vi "CreateMeanderMask_3d.vi"(7 "Rep. Rate (Hz)":dbl=10.0 min=0.0 max=34.0, 10 "Start Position":dbl[](array[numeric]) min=0.0 max=34.0) -> (0 "Laser_Ctrl":bool, 1 "start/end points":cluster{dbl, dbl, dbl}[][](array[cluster]), 2 "Canceled":bool, 5 "ImageParameter":T1)   [LabVIEW 2013]
uses:
  ImagingMS/ImageConvPara.ctl
panel:
  in  "Z Steps":i32=1 min=0 max=34
  in  "Z StepWidth":dbl=0.0001 min=0.0 max=34.0
  in  "Apply":bool
  in  "X StepWidth":dbl=0.025 min=0.0 max=34.0
  in  "Imaging?":bool=TRUE
  out "Estimated Time (min)":dbl min=0.0 max=34.0
  in  "Average/pixel":i32=10 min=0 max=34
  in  "Cancel":bool
  in  "Run":bool
  out "XY Graph":cluster{dbl, dbl, "X StepWidth":dbl}[](graph)
  out "Y Size (mm)":dbl min=0.0 max=34.0
  out "X Size (mm)":dbl min=0.0 max=34.0
  in  "Y Steps":i32=64 min=0 max=34
  in  "X Steps":i32=128 min=0 max=34
  in  "Y StepWidth":dbl=0.025 min=0.0 max=34.0
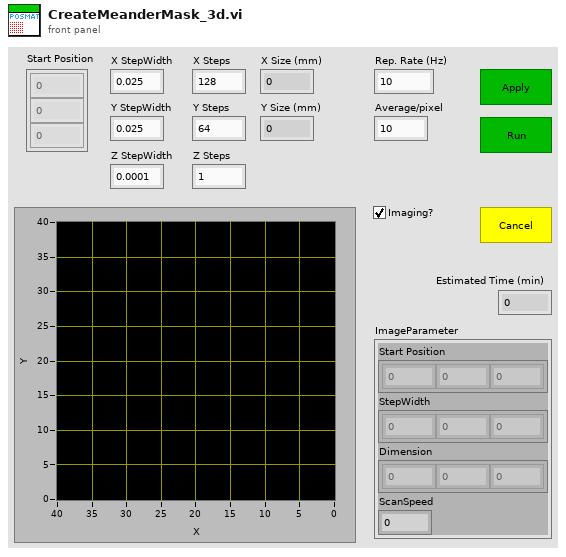
[diagram p1: front panel]
types:
  T1 = typedef "ImageConvPara.ctl" = cluster{"Start Position":dbl[], "StepWidth":dbl[], "Dimension":i32[], "ScanSpeed":dbl}
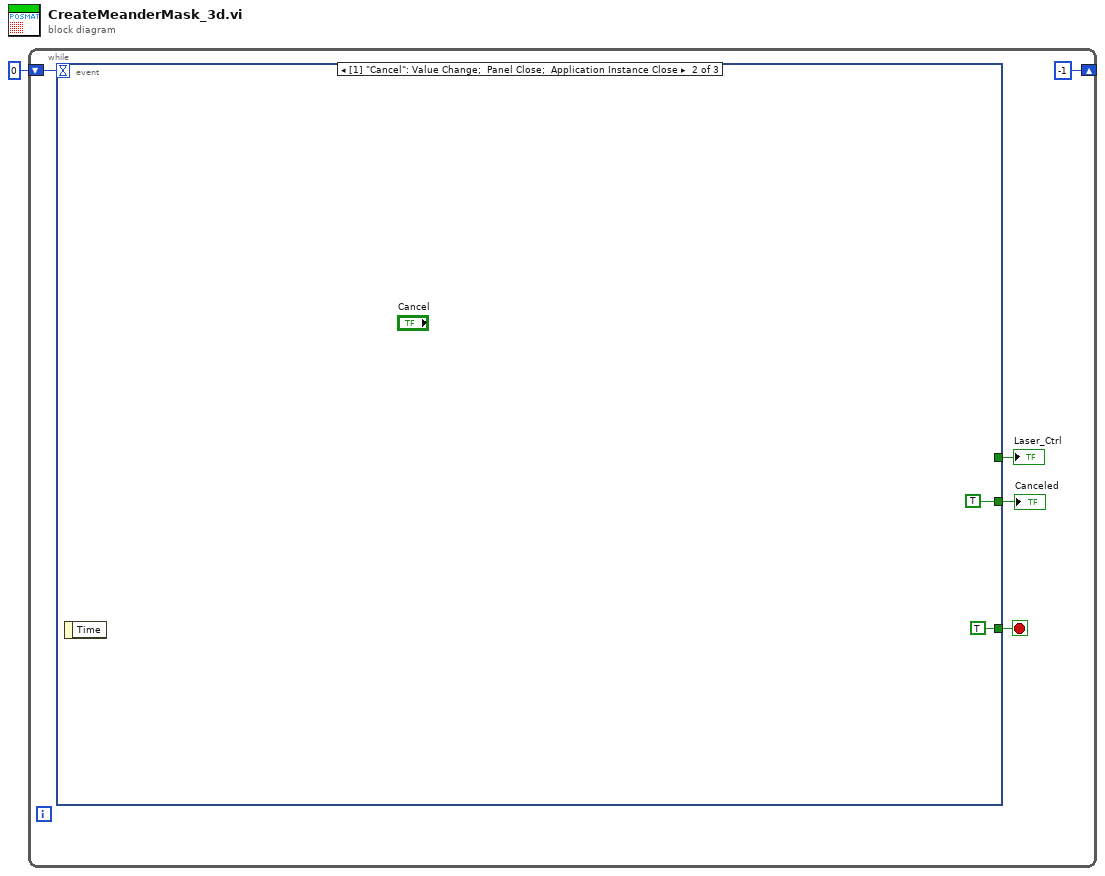
[diagram p0: block diagram]
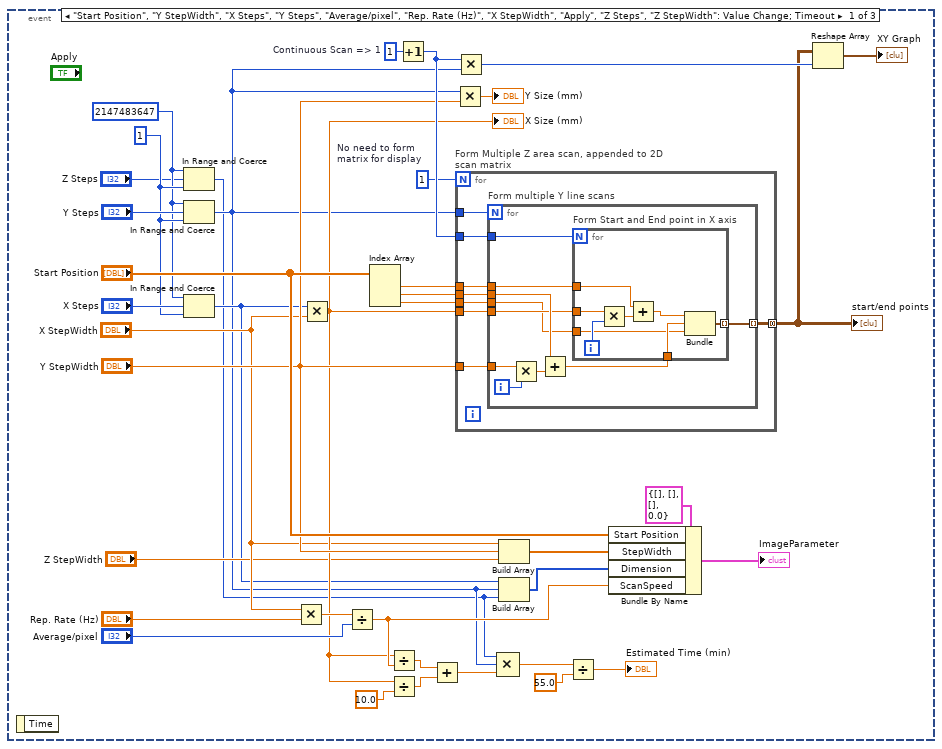
[diagram p2: hidden frame]
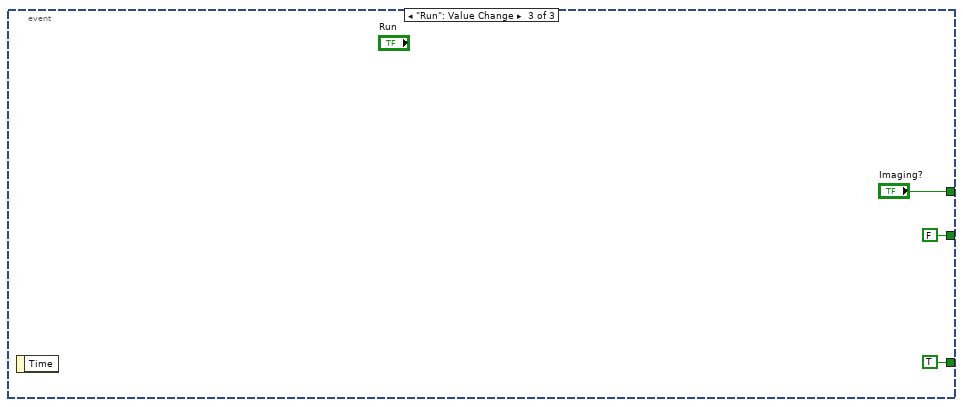
[diagram p3: hidden frame]
diagram:
  n1 = while {
    shift-right: [-1] -> _
    shift-left: 0 -> [w3]
    stop <- w6 stop-if-true
    n2 = event shown="[1] \"Cancel\": Value Change;  Panel Close;  Application Instance Close" {
      selector: _ -> [_ _ _]
      dyn-events: _ -> [_ _ _]
      timeout: w3 -> [_ _ _]
      tunnel: [_ TRUE TRUE] -> w6
      tunnel: [_ TRUE ("Canceled") FALSE ("Canceled")] -> w5
      tunnel: [_ _ "Imaging?"] -> w4
      event "Start Position", "Y StepWidth", "X Steps", "Y Steps", "Average/pixel", "Rep. Rate (Hz)", "X StepWidth", "Apply", "Z Steps", "Z StepWidth": Value Change; Timeout {
        w9 = 1  # No need to form  matrix for display
        w13 = 2147483647 ("upper limit")
        w14 = 1 ("lower limit")
        w39 = 1  # Continuous Scan => 1
        n3 = event-data() -> ()  [unwired: 1 in, 1 out]
        n4 = In Range and Coerce(upper limit=w13, x="Z Steps", lower limit=w14) -> (coerced(x)=w7:i32)  [unwired: 1 out]
        n5 = In Range and Coerce(upper limit=w13, x="Y Steps", lower limit=w14) -> (coerced(x)=w8:i32)  [unwired: 1 out]
        n6 = In Range and Coerce(upper limit=w13, x="X Steps", lower limit=w14) -> (coerced(x)=w10:i32)  [unwired: 1 out]
        n7 = Multiply(x="X StepWidth", y="Rep. Rate (Hz)") -> (x*y=w31:dbl)
        n8 = Multiply(x=w10, y="X StepWidth") -> (x*y=w16:dbl)
        "X Size (mm)" <- w16
        n9 = Divide(x=w31, y="Average/pixel") -> (x/y=w27:dbl)
        n10 = Index Array(array="Start Position") -> (element #1=w44:dbl, element #2=w43:dbl, element #3=w18:dbl)  [unwired: 3 in]
        n11 = Divide(x=w16, y=w27) -> (x/y=w25:dbl)
        n12 = Divide(x=w16, y=10.0) -> (x/y=w24:dbl)
        n13 = Increment ("Start and end point")(x=w39) -> (x+1=w40:i32)
        n14 = Add(x=w25, y=w24) -> (x+y=w23:dbl)
        n15 = Multiply(x=w8, y="Y StepWidth") -> (x*y=→"Y Size (mm)":dbl)
        n16 = Multiply(x=w40, y=w8) -> (x*y=w41:i32)
        n17 = for "Form Multiple Z area scan, appended to 2D scan matrix" {
          N: w9 -> [_]
          tunnel: w44 -> [w52]
          tunnel: w43 -> [w51]
          tunnel: w40 -> [w50]
          tunnel: [w49] -> w37 mode=concatenating
          tunnel: "Y StepWidth" -> [w48]
          tunnel: w18 -> [w47]
          tunnel: w8 -> [w46]
          tunnel: w16 -> [w45]
          n18 = for "Form multiple Y line scans" {
            N: w46 -> [_]
            tunnel: w51 -> [w57]
            tunnel: w48 -> [w53]
            tunnel: w45 -> [w56]
            tunnel: w50 -> [w59]
            tunnel: [w58] -> w49 mode=indexing
            tunnel: w47 -> [w54]
            tunnel: w52 -> [w55]
            i -> [w62]
            n19 = Multiply(x=w53, y=w62) -> (x*y=w61:dbl)
            n20 = Add(x=w57, y=w61) -> (x+y=w60:dbl)
            n21 = for "Form Start and End point in X axis" {
              N: w59 -> [_]
              tunnel: w56 -> [w68]
              tunnel: w55 -> [w63]
              tunnel: w60 -> [w66]
              tunnel: [w67] -> w58 mode=indexing
              tunnel: w54 -> [w64]
              i -> [w69]
              n22 = Multiply(x=w68, y=w69) -> (x*y=w70:dbl)
              n23 = Add(x=w63, y=w70) -> (x+y=w65:dbl)
              n24 = Bundle(w65, w66, "X StepWidth"=w64) -> (w67:cluster{dbl, dbl, "X StepWidth":dbl})  [unwired: 1 in]
            }
          }
        }
        "start/end points" <- w37
        n25 = Compound Arithmetic op=MULTIPLY(w7, w8, w23) -> (w22:dbl)
        n26 = Build Array("X StepWidth", "Y StepWidth", "Z StepWidth") -> (w34:dbl[])
        n27 = Build Array(w10, w8, w7) -> (w33:i32[])
        n28 = Divide(x=w22, y=55.0) -> (x/y=→"Estimated Time (min)":dbl)
        n29 = Bundle By Name(cluster=T1 {"Start Position"=[], "StepWidth"=[], "Dimension"=[], "ScanSpeed"=0.0} ("ImageParameter"), "Start Position"="Start Position", "StepWidth"=w34, "Dimension"=w33, "ScanSpeed"=w27) -> (→"ImageParameter":T1)
        n30 = Reshape Array(w37, w41) -> (→"XY Graph":cluster{dbl, dbl, "X StepWidth":dbl}[])
      }
      event "Cancel": Value Change; Panel Close; Application Instance Close {
        n31 = event-data() -> ()  [unwired: 1 in, 1 out]
      }
      event "Run": Value Change {
        n32 = event-data() -> ()  [unwired: 1 in, 1 out]
      }
    }
    "Canceled" <- w5
    "Laser_Ctrl" <- w4
  }
